vi "Build_Asylum_SetInWavePair.vi"(4 "decimation":i32, 6 "callback":string, 7 "whichBank":i32, 8 "error in (no error)":errorcluster, 9 "WaveB":cluster{"channelStringB":string, "waveB":string}, 10 "WaveA":cluster{"channelStringA":string, "waveA":string}, 11 "eventString":string) -> (0 "error out":errorcluster, 3 "Command":string)   [LabVIEW 2019]
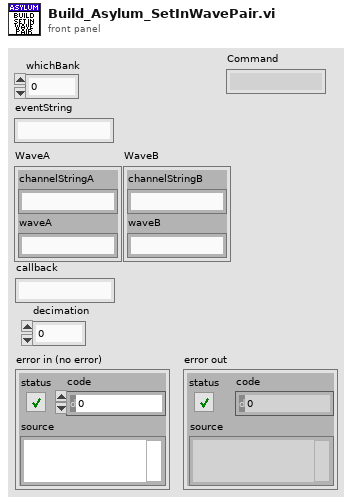
[diagram p1: front panel]
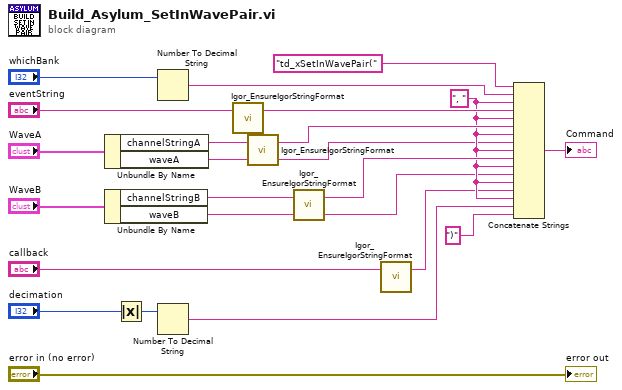
[diagram p0: block diagram]
diagram:
  w9 = ", "
  n1 = Unbundle By Name("WaveA") -> ("channelStringA"=w22:string, "waveA"=w4:string)
  n2 = Unbundle By Name("WaveB") -> ("channelStringB"=w13:string, "waveB"=w5:string)
  n3 = Absolute Value(x="decimation") -> (abs(x)=w21:i32)
  n4 = Number To Decimal String(number="whichBank") -> (decimal integer string=w19:string)  [unwired: 1 in]
  n5 = Number To Decimal String(number=w21) -> (decimal integer string=w8:string)  [unwired: 1 in]
  n6 = call <userlib>:"Igor_EnsureIgorStringFormat.vi"("Value"="eventString") -> ("Value"=w18:string)  [unwired: 2 in]
  n7 = call <userlib>:"Igor_EnsureIgorStringFormat.vi"("Value"=w22) -> ("Value"=w17:string)  [unwired: 2 in]
  n8 = call <userlib>:"Igor_EnsureIgorStringFormat.vi"("Value"=w13) -> ("Value"=w10:string)  [unwired: 2 in]
  n9 = call <userlib>:"Igor_EnsureIgorStringFormat.vi"("Value"="callback") -> ("Value"=w2:string)  [unwired: 2 in]
  n10 = Concatenate Strings("td_xSetInWavePair(" ("string"), w19, w9, w18, w9, w17, w9, w4, w9, w10, w9, w5, w9, w2, w9, w8, ")" ("string")) -> (→"Command":string)
  "error out" <- "error in (no error)"
